vi "Get MB HR and Coils.vi"() -> (2 "MB Coils":T1[](array[typedef]), 3 "MB Holding Register":T1[](array[typedef]))   [LabVIEW 2021]
uses:
  Modbus Address Cluster.ctl
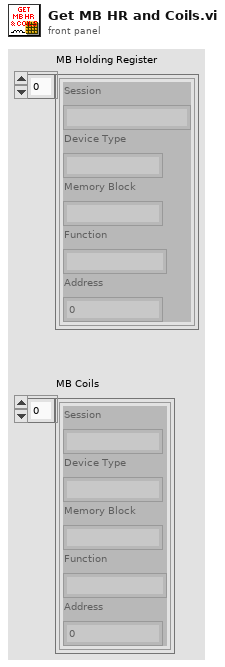
[diagram p1: front panel]
types:
  T1 = typedef "Modbus Address Cluster.ctl" = cluster{"Session":string, "Device Type":string, "Memory Block":string, "Function":string, "Address":u16}
  T2 = typedef "Device Settings.ctl" = cluster{"Session":string, "Key and Value":string[][]}
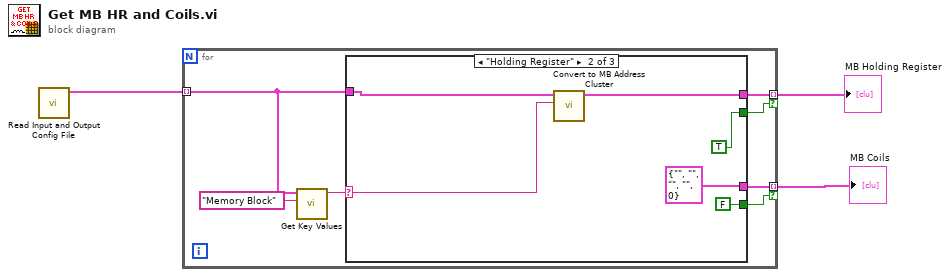
[diagram p0: block diagram]
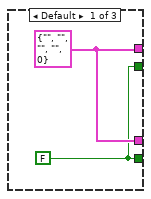
[diagram p2: hidden frame]
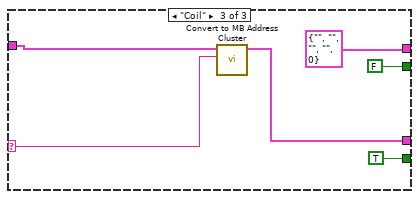
[diagram p3: hidden frame]
diagram:
  n1 = call "Read Input and Output Config File.vi"() -> ("Input and Output Settings"=w2:T2[])  [unwired: 10 in, 1 out]
  n2 = for {
    tunnel: w2 -> [w9] mode=indexing
    tunnel: [w8] -> w3 mode=indexing if=w7
    tunnel: [w5] -> w1 mode=indexing if=w4
    n3 = call "Get Key Values.vi"("Search Key"="Memory Block" ("key"), "Configure Cluster"=w9) -> ("value"=w10:string)  [unwired: 8 in, 1 out]
    n4 = case shown="\"Holding Register\"" w10 {
      selector: w10 -> [_ w17 w23]
      tunnel: w9 -> [_ w16 w22]
      tunnel: [w12 w15 T1 {"Session"="", "Device Type"="", "Memory Block"="", "Function"="", "Address"=0} ("Modbus Input/output cluster")] -> w8
      tunnel: [w11 TRUE FALSE] -> w7
      tunnel: [w12 T1 {"Session"="", "Device Type"="", "Memory Block"="", "Function"="", "Address"=0} ("Modbus Input/output cluster") w20] -> w5
      tunnel: [w11 FALSE TRUE] -> w4
      frame Default {
        w12 = T1 {"Session"="", "Device Type"="", "Memory Block"="", "Function"="", "Address"=0}
        w11 = FALSE
      }
      frame "Holding Register" {
        n5 = call "Convert to MB Address Cluster.vi"("String"=w17, "Device Settings"=w16) -> ("Modbus Input/output cluster"=w15:T1)  [unwired: 9 in]
      }
      frame "Coil" {
        n6 = call "Convert to MB Address Cluster.vi"("String"=w23, "Device Settings"=w22) -> ("Modbus Input/output cluster"=w20:T1)  [unwired: 9 in]
      }
    }
  }
  "MB Holding Register" <- w3
  "MB Coils" <- w1
